vi "Define DataGrid Columns.vi"(8 "error in (no error)":errorcluster, 10 "ColumnSetup":T1[](array[typedef]) {"MinWidth" min=2 step=1; "AutoSizeMode" items=["None"=1, "ColumnHeader"=2, "AllCellsExceptHeader"=4, "AllCells"=6, "DisplayedCellsExceptHeader"=8, "DisplayedCells"=10, "Fill"=16]; "FillWeight" min=1 max=100}, 11 "DataGrid in":refnum<class "DataGridView.lvclass">) -> (0 "error out":errorcluster, 2 "ColumnDefs":refnum<class "GridColumn.lvclass">[](array[class]), 3 "DataGrid out":refnum<class "DataGridView.lvclass">)   [LabVIEW 2013, in "DataGrid.lvlib" / "DataGridView.lvclass"]
doc: "Defines the columns of the dataTable that is used to store all display data. If called more than once, it will add columns to the existing dataTable, so resulting in more (possibly duplicate) columns."
uses:
  DataGridView.lvclass
  GridColumn/ColumnDefinition.ctl
  GridColumn/ColumnType.ctl
  GridColumn/GridColumn.lvclass
  DataGridView.lvclass/DataGridView.ctl
  System.Windows.Forms
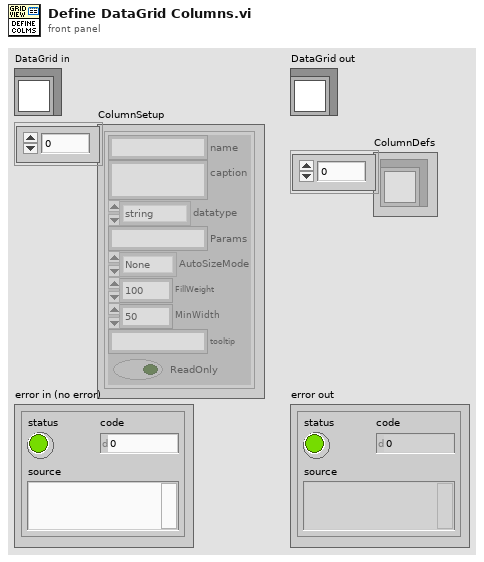
[diagram p1: front panel]
types:
  T1 = typedef "DataGrid.lvlib/GridColumn.lvclass/ColumnDefinition.ctl" = cluster{"name":string, "caption":string, "datatype":T2, "Params":string, "AutoSizeMode":i32, "FillWeight":sgl, "MinWidth":u32, "tooltip":string, "ReadOnly":bool}
  T2 = typedef "DataGrid.lvlib/GridColumn.lvclass/ColumnType.ctl" = enum16{"string", "image", "check", "numeric", "timestamp", "button", "combo", "link"}
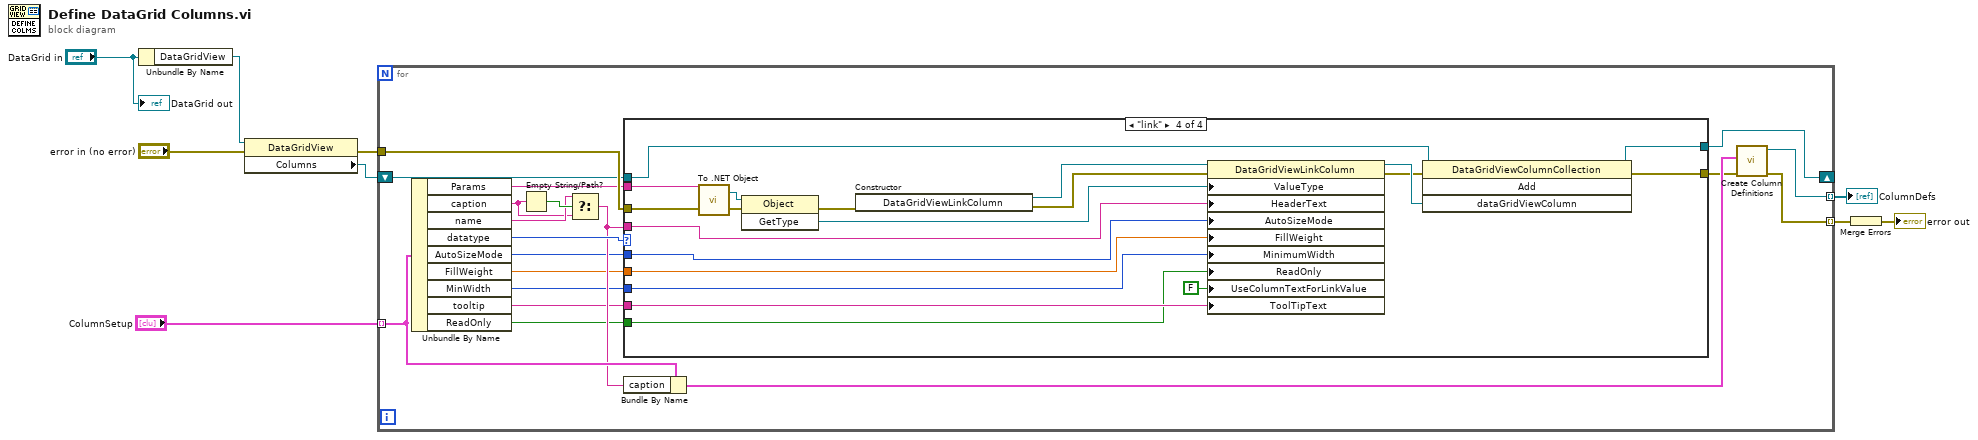
[diagram p0: block diagram]
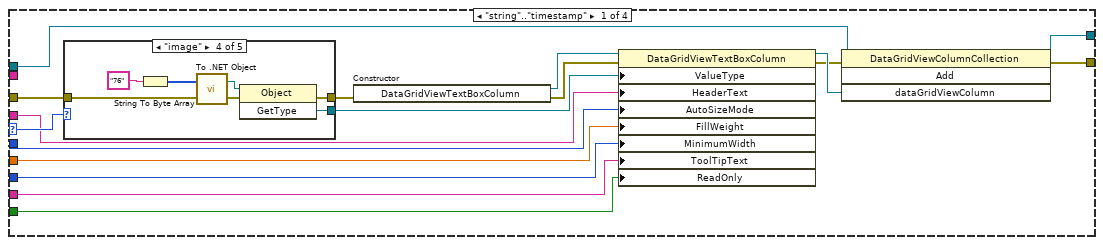
[diagram p2: hidden frame]
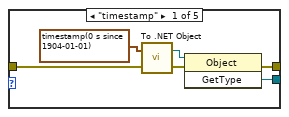
[diagram p3: hidden frame]
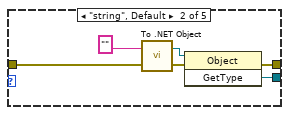
[diagram p4: hidden frame]
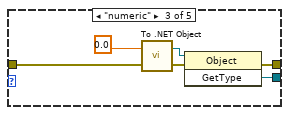
[diagram p5: hidden frame]
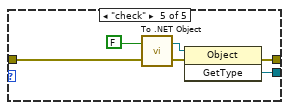
[diagram p6: hidden frame]
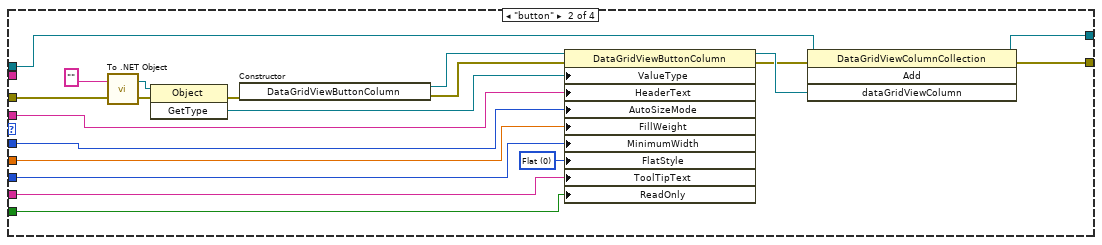
[diagram p7: hidden frame]
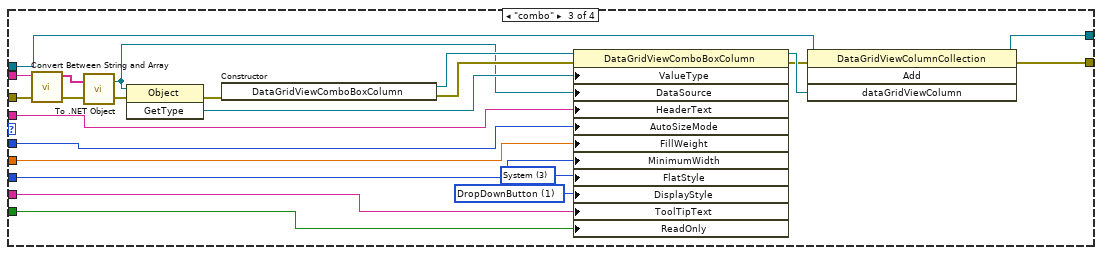
[diagram p8: hidden frame]
diagram:
  n1 = Unbundle By Name("DataGrid in") -> ("DataGridView"=w4:refnum<k24>)
  n2 = property class="DataGridView"(reference=w4, error in="error in (no error)") -> (error out=w2:errorcluster, "Columns"=w5:refnum<k24>)  [unwired: 1 out]
  n3 = for {
    tunnel: "ColumnSetup" -> [w23] mode=indexing
    tunnel: [w13] -> w7 mode=indexing
    shift-right: [w14] -> _
    shift-left: w5 -> [w15]
    tunnel: [w27] -> w6 mode=indexing
    tunnel: w2 -> [w26]
    n4 = Unbundle By Name(w23) -> ("Params"=w12:string, "caption"=w21:string, "name"=w24:string, "datatype"=w28:T2, "AutoSizeMode"=w17:i32, "FillWeight"=w18:sgl, "MinWidth"=w19:u32, "tooltip"=w11:string, "ReadOnly"=w10:bool)
    n5 = Empty String/Path?(string/path=w21) -> (empty?=w25:bool)
    n6 = Select(t=w24, s=w25, f=w21) -> (s? t:f=w20:string)
    n7 = case shown="\"link\"" w28 {
      selector: w28 -> [w37 _ _ _]
      tunnel: [w34 w82 w107 w126] -> w16
      tunnel: w26 -> [w45 w96 w118 w138]
      tunnel: w20 -> [w32 w79 w104 w123]
      tunnel: w19 -> [w44 w95 w117 w137]
      tunnel: w18 -> [w43 w94 w116 w136]
      tunnel: w17 -> [w42 w93 w115 w135]
      tunnel: w15 -> [w31 w81 w106 w125]
      tunnel: [w33 w80 w105 w124] -> w14
      tunnel: w12 -> [_ _ w103 w121]
      tunnel: w11 -> [w30 w78 w98 w120]
      tunnel: w10 -> [w29 w77 w97 w119]
      frame "string".."timestamp" {
        n8 = case shown="\"image\"" w37 {
          tunnel: w45 -> [w49 w55 w61 w68 w74]
          tunnel: [w48 w54 w60 w67 w73] -> w40
          tunnel: [w47 w53 w59 w66 w72] -> w38
          frame "timestamp" {
            n9 = call <vilib>:"To .NET Object.vi"("error in (no error)"=w49, "anything"=timestamp(0 s since 1904-01-01) ("name")) -> ("error out"=w50:errorcluster, ".NET object"=w51:refnum<k24>)
            n10 = invoke class="Object" method="GetType"(reference=w51, error in=w50) -> (error out=w47:errorcluster, "GetType"=w48:refnum<k24>)  [unwired: 1 in, 1 out]
          }
          frame "string", Default {
            n11 = call <vilib>:"To .NET Object.vi"("error in (no error)"=w55, "anything"="") -> ("error out"=w56:errorcluster, ".NET object"=w57:refnum<k24>)
            n12 = invoke class="Object" method="GetType"(reference=w57, error in=w56) -> (error out=w53:errorcluster, "GetType"=w54:refnum<k24>)  [unwired: 1 in, 1 out]
          }
          frame "numeric" {
            n13 = call <vilib>:"To .NET Object.vi"("error in (no error)"=w61, "anything"=0.0) -> ("error out"=w62:errorcluster, ".NET object"=w63:refnum<k24>)
            n14 = invoke class="Object" method="GetType"(reference=w63, error in=w62) -> (error out=w59:errorcluster, "GetType"=w60:refnum<k24>)  [unwired: 1 in, 1 out]
          }
          frame "image" {
            n15 = String To Byte Array(string="76") -> (unsigned byte array=w64:u8[])
            n16 = call <vilib>:"To .NET Object.vi"("error in (no error)"=w68, "anything"=w64) -> ("error out"=w69:errorcluster, ".NET object"=w70:refnum<k24>)
            n17 = invoke class="Object" method="GetType"(reference=w70, error in=w69) -> (error out=w66:errorcluster, "GetType"=w67:refnum<k24>)  [unwired: 1 in, 1 out]
          }
          frame "check" {
            n18 = call <vilib>:"To .NET Object.vi"("error in (no error)"=w74, "anything"=FALSE) -> ("error out"=w75:errorcluster, ".NET object"=w76:refnum<k24>)
            n19 = invoke class="Object" method="GetType"(reference=w76, error in=w75) -> (error out=w72:errorcluster, "GetType"=w73:refnum<k24>)  [unwired: 1 in, 1 out]
          }
        }
        n20 = constructor class="DataGridViewTextBoxColumn"(error in=w38) -> (reference out=w41:refnum<k24>, error out=w39:errorcluster)  [unwired: 2 in, 1 out]
        n21 = property class="DataGridViewTextBoxColumn"(reference=w41, error in=w39, "ValueType"=w40, "HeaderText"=w32, "AutoSizeMode"=w42, "FillWeight"=w43, "MinimumWidth"=w44, "ToolTipText"=w30, "ReadOnly"=w29) -> (reference out=w36:refnum<k24>, error out=w35:errorcluster)
        n22 = invoke class="DataGridViewColumnCollection" method="Add"(reference=w31, error in=w35, "dataGridViewColumn"=w36) -> (reference out=w33:refnum<k24>, error out=w34:errorcluster)  [unwired: 1 in, 2 out]
      }
      frame "button" {
        w85 = 0 items=["Flat", "Popup", "Standard", "System"] ("FlatStyle")
        n23 = call <vilib>:"To .NET Object.vi"("error in (no error)"=w96, "anything"="") -> ("error out"=w88:errorcluster, ".NET object"=w89:refnum<k24>)
        n24 = invoke class="Object" method="GetType"(reference=w89, error in=w88) -> (error out=w91:errorcluster, "GetType"=w92:refnum<k24>)  [unwired: 1 in, 1 out]
        n25 = constructor class="DataGridViewButtonColumn"(error in=w91) -> (reference out=w86:refnum<k24>, error out=w90:errorcluster)  [unwired: 2 in, 1 out]
        n26 = property class="DataGridViewButtonColumn"(reference=w86, error in=w90, "ValueType"=w92, "HeaderText"=w79, "AutoSizeMode"=w93, "FillWeight"=w94, "MinimumWidth"=w95, "FlatStyle"=w85, "ToolTipText"=w78, "ReadOnly"=w77) -> (reference out=w84:refnum<k24>, error out=w83:errorcluster)
        n27 = invoke class="DataGridViewColumnCollection" method="Add"(reference=w81, error in=w83, "dataGridViewColumn"=w84) -> (reference out=w80:refnum<k24>, error out=w82:errorcluster)  [unwired: 1 in, 2 out]
      }
      frame "combo" {
        w101 = 1 items=["ComboBox", "DropDownButton", "Nothing"] ("DisplayStyle")
        w110 = 3 items=["Flat", "Popup", "Standard", "System"] ("FlatStyle")
        n28 = call "Convert Between String and Array.vi"("String"=w103) -> ("String Array"=w102:string[])  [unwired: 9 in, 1 out]
        n29 = call <vilib>:"To .NET Object.vi"("error in (no error)"=w118, "anything"=w102) -> ("error out"=w112:errorcluster, ".NET object"=w99:refnum<k24>)
        n30 = invoke class="Object" method="GetType"(reference=w99, error in=w112) -> (error out=w114:errorcluster, "GetType"=w100:refnum<k24>)  [unwired: 1 in, 1 out]
        n31 = constructor class="DataGridViewComboBoxColumn"(error in=w114) -> (reference out=w111:refnum<k24>, error out=w113:errorcluster)  [unwired: 2 in, 1 out]
        n32 = property class="DataGridViewComboBoxColumn"(reference=w111, error in=w113, "ValueType"=w100, "DataSource"=w99, "HeaderText"=w104, "AutoSizeMode"=w115, "FillWeight"=w116, "MinimumWidth"=w117, "FlatStyle"=w110, "DisplayStyle"=w101, "ToolTipText"=w98, "ReadOnly"=w97) -> (reference out=w109:refnum<k24>, error out=w108:errorcluster)
        n33 = invoke class="DataGridViewColumnCollection" method="Add"(reference=w106, error in=w108, "dataGridViewColumn"=w109) -> (reference out=w105:refnum<k24>, error out=w107:errorcluster)  [unwired: 1 in, 2 out]
      }
      frame "link" {
        n34 = call <vilib>:"To .NET Object.vi"("error in (no error)"=w138, "anything"=w121) -> ("error out"=w130:errorcluster, ".NET object"=w131:refnum<k24>)
        n35 = invoke class="Object" method="GetType"(reference=w131, error in=w130) -> (error out=w133:errorcluster, "GetType"=w134:refnum<k24>)  [unwired: 1 in, 1 out]
        n36 = constructor class="DataGridViewLinkColumn"(error in=w133) -> (reference out=w129:refnum<k24>, error out=w132:errorcluster)  [unwired: 2 in, 1 out]
        n37 = property class="DataGridViewLinkColumn"(reference=w129, error in=w132, "ValueType"=w134, "HeaderText"=w123, "AutoSizeMode"=w135, "FillWeight"=w136, "MinimumWidth"=w137, "ReadOnly"=w119, "UseColumnTextForLinkValue"=FALSE, "ToolTipText"=w120) -> (reference out=w128:refnum<k24>, error out=w127:errorcluster)
        n38 = invoke class="DataGridViewColumnCollection" method="Add"(reference=w125, error in=w127, "dataGridViewColumn"=w128) -> (reference out=w124:refnum<k24>, error out=w126:errorcluster)  [unwired: 1 in, 2 out]
      }
    }
    n39 = Bundle By Name(cluster=w23, "caption"=w20) -> (w22:T1)
    n40 = call "Create Column Definitions.vi"("error in (no error)"=w16, "Column"=w22) -> ("error out"=w13:errorcluster, "GridColumn out"=w27:refnum<class "GridColumn.lvclass">)  [unwired: 8 in]
  }
  "ColumnDefs" <- w6
  n41 = Merge Errors(w7) -> (→"error out":errorcluster)
  "DataGrid out" <- "DataGrid in"
